vi "1_Sin(x)(Training).vi"() -> ()   [LabVIEW 2020]
uses:
  <vilib>/Ngene/Deep Learning Toolkit/Toolkit/NN_Train/Controls/NN_Train_Params.ctl
  <vilib>/Ngene/Deep Learning Toolkit/Toolkit/NN_Train/Controls/NN_Train_Optimizer.ctl
  <vilib>/Ngene/Deep Learning Toolkit/Toolkit/NN_Train/Controls/NN_Train_Data_Sampling.ctl
  <vilib>/Ngene/Deep Learning Toolkit/Toolkit/NN_Train/Controls/NN_LR_Policy_Cfg.ctl
  <vilib>/Ngene/Deep Learning Toolkit/Toolkit/NN_Train/Controls/NN_LR_Policy_Type.ctl
  <vilib>/Ngene/Deep Learning Toolkit/Toolkit/NN_Train/Controls/NN_Train_Session_Data.ctl
  <vilib>/Ngene/Deep Learning Toolkit/Toolkit/NN_Layers/Layers/Input/Controls/NN_Layer_Config(Input1D).ctl
  <vilib>/Ngene/Deep Learning Toolkit/Toolkit/NN_Data/Controls/NN_Data_type.ctl
  <vilib>/Ngene/Deep Learning Toolkit/Toolkit/NN_Network/Controls/NN_Save_Before_Destroy_Options.ctl
  <vilib>/Ngene/Deep Learning Toolkit/Toolkit/NN_Network/Controls/NN_Device.ctl
  <vilib>/Ngene/Deep Learning Toolkit/Toolkit/NN_Layers/Layers/FC/Controls/NN_Layer_Config(FC).ctl
  <vilib>/Ngene/Deep Learning Toolkit/Toolkit/NN_Layers/Layers/BatchNorm/Controls/NN_BN_Params.ctl
  <vilib>/Ngene/Deep Learning Toolkit/Toolkit/NN_Activations/Controls/NN_Activation_Type.ctl
  <vilib>/Ngene/Deep Learning Toolkit/Toolkit/NN_Layers/Controls/NN_Layer_Init_Params.ctl
  <vilib>/Ngene/Deep Learning Toolkit/Toolkit/NN_Layers/Controls/NN_Layer_Weight_Init_Type.ctl
  <vilib>/Ngene/Deep Learning Toolkit/Toolkit/NN_Data/API/DataSet/DataSet_Types/NN_DataSet(In1D_Out1D).ctl
  <vilib>/Ngene/Deep Learning Toolkit/Toolkit/NN_Data/Controls/DataRef_Types/2D/NN_Data_ref(2D_SGL).ctl
  <vilib>/Analysis/1siggen.llb/Ramp Pattern by Samples.vi
  <vilib>/Ngene/Deep Learning Toolkit/Toolkit/NN_Layers/Layers/Input/NN_Layer_Create(Input1D).vi
  <vilib>/Ngene/Deep Learning Toolkit/Toolkit/NN_Layers/Layers/FC/NN_Layer_Create(FC).vi
  <vilib>/Ngene/Deep Learning Toolkit/Toolkit/NN_Train/Loss_Functions/NN_Set_Loss(MSE).vi
  <vilib>/Ngene/Deep Learning Toolkit/Toolkit/NN_Data/subVIs/Get_Data_Vals/2D/NN_Data_Get_ValByRef(2D_SGL).vi
  <vilib>/Ngene/Deep Learning Toolkit/Toolkit/NN_Network/subVIs/NN_Predict/NN_Predict(In1D_Out1D).vi
  <vilib>/Ngene/Deep Learning Toolkit/Toolkit/NN_Train/Eval_Loss/NN_Eval_Test_Error_Loss/NN_Eval(In1D_Out1D).vi
  <vilib>/Ngene/Deep Learning Toolkit/Toolkit/Deep_Learning_Toolkit_by_Ngene.lvlib
  <vilib>/Analysis/NI_AALBase.lvlib
panel:
  out "Loop Time":dbl=0.0014889000000266606 format="%#_4p"
  out "Test Loss":sgl=6.473779e-05
  out "Training Loss":sgl=6.795796e-05
  in  "Stop":bool
  out "Loss Chart":cluster{"Loss":sgl, "Test Loss":sgl}(graph)={"Loss"=6.795796e-05, "Test Loss"=6.473779e-05}
  in  "# of Sine Cycles":dbl=4.0
  out "Sin(x): Predictions vs Ground Truths":sgl[][](graph)
  in  "Eval?":bool
  out "Session Data":T1={"Epochs"=1922.368, "Tot_Iter"=30037, "LR"=1.953125e-05, "LR_iter"=30038}
  in  "LR_Decay_Params":T2={"Policy_Type"=enum."Step", "LR0"=0.01, "k"=200.0, "WarmUp_Policy"=enum."Ramp", "WarmUp_Iter"=100, "WarmUp_Ratio"=10.0} {"WarmUp_Ratio" min=1; "WarmUp_Iter" min=1; "LR0" format="%.7f"}
  in  "NN_Train_Params":T4={"Optimizer"=enum."Adam", "Beta_1"=0.9, "Beta_2"=0.999, "Weight Decay(L1)"=1e-08, "Weight Decay(L2)"=1e-08, "Data_Sampling"=enum."Random"}
  # "Overview: Demonstrates the usage of DeepLTK (Deep Learning Toolkit for LabVIEW) for solving a simple regression problem of modeling sin(x) function.\nRequirements: DeepLTK - Deep Learning Toolkit for LabVIEW (https://www.ngene.co/deep-learning-toolkit-for-labview)\nInstructions:\n1. Run the VI with default configurations.\n2. Observe how the training loss is decreasing.\n3. Periodically press \"Eval?\" button to observe \"Test Loss\" and performance of the model on Test Dataset\n4. Press \"Stop\" when \"Test Loss\" is is not decreasing. ~1500 epochs\nMore Examples:  https://github.com/ngenehub/deepltk_examples"
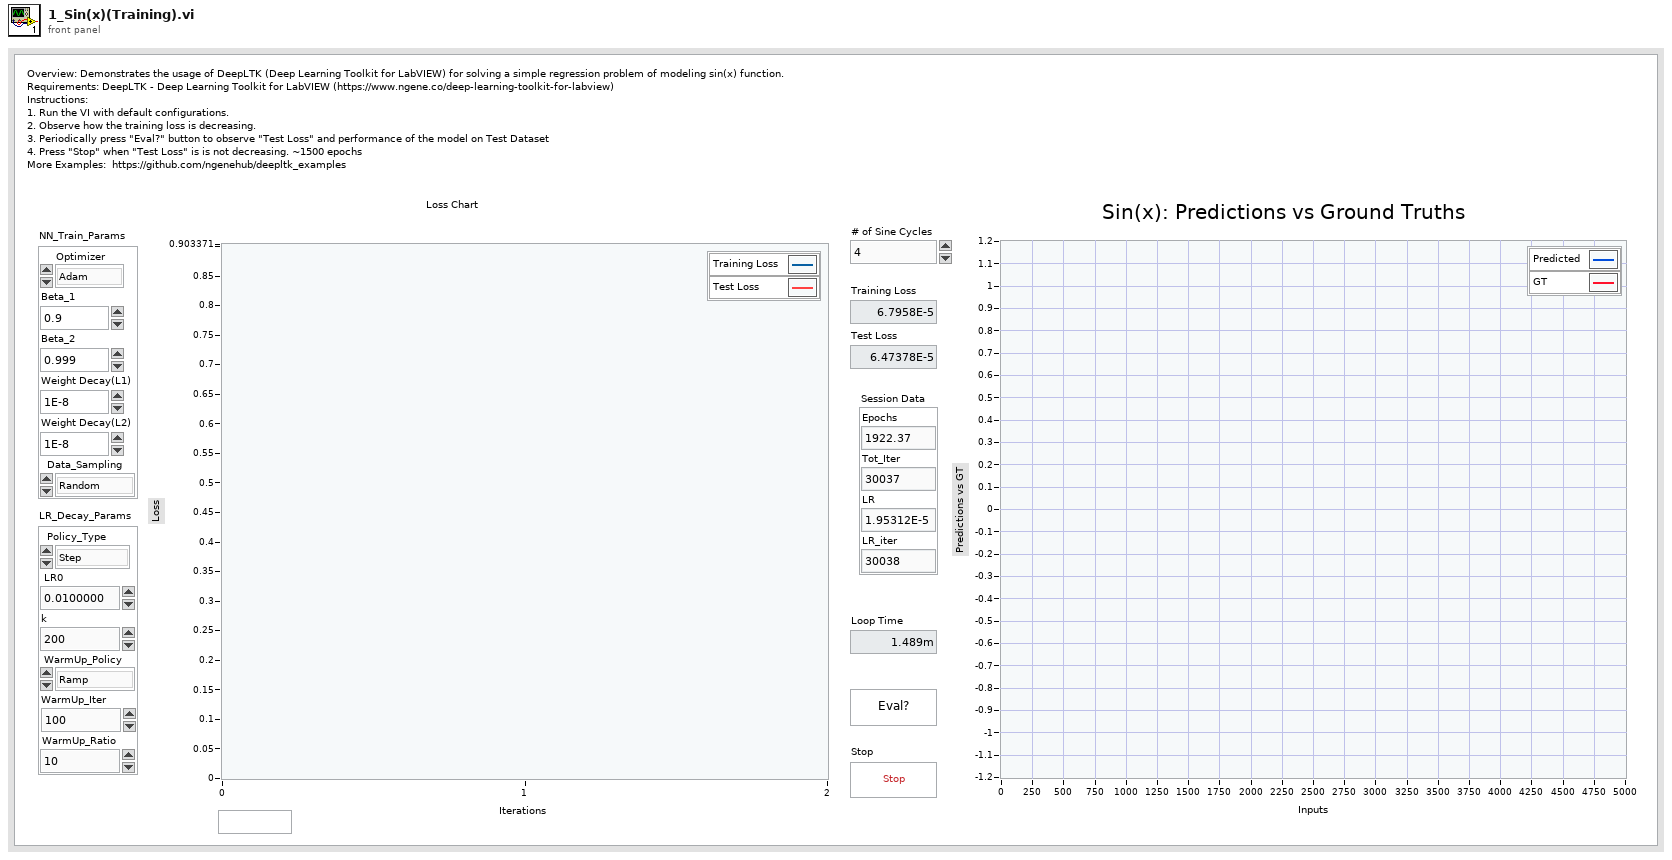
[diagram p1: front panel]
types:
  T1 = typedef "Deep_Learning_Toolkit_by_Ngene.lvlib/NN_Train_Session_Data.ctl" = cluster{"Epochs":sgl, "Tot_Iter":i32, "LR":sgl, "LR_iter":i32}
  T2 = typedef "Deep_Learning_Toolkit_by_Ngene.lvlib/NN_LR_Policy_Cfg.ctl" = cluster{"Policy_Type":T3, "LR0":dbl, "k":sgl, "WarmUp_Policy":enum16{"Step", "Ramp"}, "WarmUp_Iter":i32, "WarmUp_Ratio":sgl}
  T3 = typedef "Deep_Learning_Toolkit_by_Ngene.lvlib/NN_LR_Policy_Type.ctl" = enum16{"Manual", "Step", "Exp", "1/t"}
  T4 = typedef "Deep_Learning_Toolkit_by_Ngene.lvlib/NN_Train_Params.ctl" = cluster{"Optimizer":T5, "Beta_1":sgl, "Beta_2":sgl, "Weight Decay(L1)":sgl, "Weight Decay(L2)":sgl, "Data_Sampling":T6}
  T5 = typedef "Deep_Learning_Toolkit_by_Ngene.lvlib/NN_Train_Optimizer.ctl" = enum16{"SGD", "Adam", "Adagrad", "Adadelta", "RMSProp", "Nesterov"}
  T6 = typedef "Deep_Learning_Toolkit_by_Ngene.lvlib/NN_Train_Data_Sampling.ctl" = enum16{"Random", "Sequential"}
  T7 = typedef "Deep_Learning_Toolkit_by_Ngene.lvlib/NN_Layer_Config(FC).ctl" = cluster{"Name":string, "Size":i32, "BN":bool, "BN_Params":T8, "Activation":T9, "Has Bias?":bool, "Init_Params":T10, "Custom_Params":string}
  T8 = typedef "Deep_Learning_Toolkit_by_Ngene.lvlib/NN_BN_Params.ctl" = cluster{"epsilon":sgl, "momentum":sgl}
  T9 = typedef "Deep_Learning_Toolkit_by_Ngene.lvlib/NN_Activation_Type.ctl" = enum16{"Sigmoid", "ReLU", "LReLU", "ReLU6", "GELU", "tanh", "Swish", "Mish", "None"}
  T10 = typedef "Deep_Learning_Toolkit_by_Ngene.lvlib/NN_Layer_Init_Params.ctl" = cluster{"Init_Type":T11, "Value":sgl}
  T11 = typedef "Deep_Learning_Toolkit_by_Ngene.lvlib/NN_Layer_Weight_Init_Type.ctl" = enum16{"Const", "Uniform", "Gaussian", "Xavier"}
  T12 = typedef "Deep_Learning_Toolkit_by_Ngene.lvlib/NN_DataSet(In1D_Out1D).ctl" = cluster{"Inputs Ref.":variant, "Outputs Ref.":T13, "Dims_In":i32, "Dataset_Size":i32, "Dims_Out":i32, "Labels":string[], "File Paths":path[], "Custom_Data":variant}
  T13 = typedef "Deep_Learning_Toolkit_by_Ngene.lvlib/NN_Data_ref(2D_SGL).ctl" = refnum<data-value>
  T14 = typedef "Deep_Learning_Toolkit_by_Ngene.lvlib/NN_Device.ctl" = enum16{"CPU", "GPU"}
  T15 = typedef "Deep_Learning_Toolkit_by_Ngene.lvlib/NN_Save_Before_Destroy_Options.ctl" = cluster{"CFG?":bool, "Weights?":bool, "Render?":bool}
  T16 = typedef "Deep_Learning_Toolkit_by_Ngene.lvlib/NN_Layer_Config(Input1D).ctl" = cluster{"Name":string, "Size":i32, "Data_Type":T17, "Shift":sgl, "Scale":sgl}
  T17 = typedef "Deep_Learning_Toolkit_by_Ngene.lvlib/NN_Data_type.ctl" = enum16{"I8", "U8", "I16", "U16", "U32 ARGB", "SGL"}
  T18 = typedef "Deep_Learning_Toolkit_by_Ngene.lvlib/NN.ctl" = cluster{"Name":string, "No of Layers":i32, "mBatch":i32, "Layers":T19[], "Dimty":T20, "Dims_In":T21, "Dims_Out":T21, "Working_Dir":path, "Train?":bool, "Train_Params":T4, "LR_Update_Policy":T2, "Session Data":T1, "Ground_truth":T22, "NNg_hdls":T23, "NN_Device":T14, "GPU Id":i32, "Labels":string[], "Loss_Type":T24, "Loss_Cfg_Prms":variant, "NNG_WS":T25, "DryRun?":bool}
  T19 = typedef "Deep_Learning_Toolkit_by_Ngene.lvlib/NN_Layer_ref.ctl" = refnum<file>
  T20 = typedef "Deep_Learning_Toolkit_by_Ngene.lvlib/NN_In_Out_Dim-ty.ctl" = enum8{"In1D_Out1D", "In3D_Out1D", "In3D_Out3D", "In3D_OutBBox"}
  T21 = typedef "Deep_Learning_Toolkit_by_Ngene.lvlib/NN_Dims(C,H,W).ctl" = cluster{"C":i32, "H":i32, "W":i32}
  T22 = typedef "Deep_Learning_Toolkit_by_Ngene.lvlib/NN_Ground_truth.ctl" = cluster{"Y":variant}
  T23 = typedef "Deep_Learning_Toolkit_by_Ngene.lvlib/nng_cuda_handles.ctl" = cluster{"cudnn":u64, "cublas":u64, "stream":u64, "curand":u64}
  T24 = typedef "Deep_Learning_Toolkit_by_Ngene.lvlib/NN_Loss_Type.ctl" = enum16{"None", "MSE", "CrossEntropy", "YOLO_v2", "YOLO_v4"}
  T25 = typedef "Deep_Learning_Toolkit_by_Ngene.lvlib/NNG_WS.ctl" = cluster{"NNG_WS_Mem":T26, "Max_WS_Size":i64}
  T26 = typedef "Deep_Learning_Toolkit_by_Ngene.lvlib/NNg_WS_Mem_DVR.ctl" = refnum<data-value>
  T27 = typedef "Deep_Learning_Toolkit_by_Ngene.lvlib/NN_Eval_Params.ctl" = cluster{"Loss":sgl, "Error":sgl}
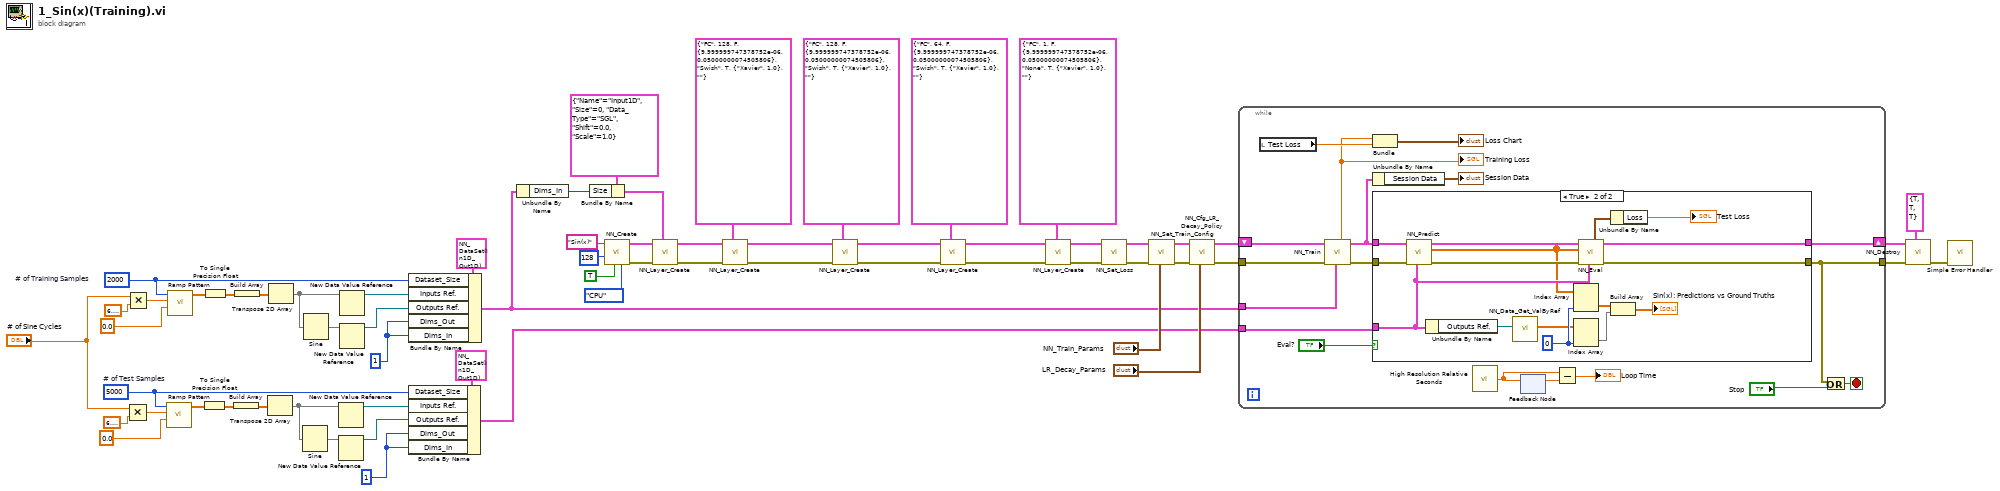
[diagram p0: block diagram]
diagram:
  w8 = 1 ("Dims_Out")
  w10 = 2000  # # of Training Samples
  w22 = 5000  # # of Test Samples
  w23 = 1 ("Dims_Out")
  n1 = Multiply(x="# of Sine Cycles", y=6.283185307179586) -> (x*y=w31:dbl)
  n2 = Multiply(x="# of Sine Cycles", y=6.283185307179586) -> (x*y=w17:dbl)
  n3 = call-poly <vilib>:"Ramp Pattern.vi"("start"=0.0, "end"=w31, "samples"=w22) -> ("Ramp Pattern"=w29:dbl[])  [unwired: 7 in, 1 out]
  n4 = call-poly <vilib>:"Ramp Pattern.vi"("start"=0.0, "end"=w17, "samples"=w10) -> ("Ramp Pattern"=w15:dbl[])  [unwired: 7 in, 1 out]
  n5 = To Single Precision Float(number=w29) -> (single precision float=w30:sgl[])
  n6 = To Single Precision Float(number=w15) -> (single precision float=w16:sgl[])
  n7 = Build Array(w30) -> (w28:sgl[][])
  n8 = Build Array(w16) -> (w14:sgl[][])
  n9 = Transpose 2D Array(2D array=w28) -> (transposed array=w27:sgl[][])
  n10 = Transpose 2D Array(2D array=w14) -> (transposed array=w13:sgl[][])
  n11 = Sine(x=w27) -> (sin(x)=w26:sgl[][])
  n12 = Sine(x=w13) -> (sin(x)=w12:sgl[][])
  n13 = New Data Value Reference(data value=w27) -> (data value reference=w34:refnum<data-value>)  [unwired: 1 in, 1 out]
  n14 = New Data Value Reference(data value=w26) -> (data value reference=w33:refnum<data-value>)  [unwired: 1 in, 1 out]
  n15 = New Data Value Reference(data value=w13) -> (data value reference=w20:refnum<data-value>)  [unwired: 1 in, 1 out]
  n16 = New Data Value Reference(data value=w12) -> (data value reference=w19:refnum<data-value>)  [unwired: 1 in, 1 out]
  n17 = Bundle By Name(cluster=T12 {"Inputs Ref."=variant(refnum<data-value> refnum), "Outputs Ref."=refnum, "Dims_In"=0, "Dataset_Size"=0, "Dims_Out"=0, "Labels"=[], "File Paths"=[], "Custom_Data"=variant} ("Dataset(In1D_Out1D)"), "Dataset_Size"=w22, "Inputs Ref."=w34, "Outputs Ref."=w33, "Dims_Out"=w23, "Dims_In"=w23) -> (w25:T12)
  n18 = Bundle By Name(cluster=T12 {"Inputs Ref."=variant(refnum<data-value> refnum), "Outputs Ref."=refnum, "Dims_In"=0, "Dataset_Size"=0, "Dims_Out"=0, "Labels"=[], "File Paths"=[], "Custom_Data"=variant} ("Dataset(In1D_Out1D)"), "Dataset_Size"=w10, "Inputs Ref."=w20, "Outputs Ref."=w19, "Dims_Out"=w8, "Dims_In"=w8) -> (w9:T12)
  n19 = Unbundle By Name(w9) -> ("Dims_In"=w40:i32)
  n20 = Bundle By Name(cluster=T16 {"Name"="Input1D", "Size"=0, "Data_Type"=enum."SGL", "Shift"=0.0, "Scale"=1.0} ("Input1D_Cfg"), "Size"=w40) -> (w56:T16)
  n21 = call <vilib>:"NN_Create.vi"("NN_Device"=NN_Device."CPU", "Train? (false)"=TRUE, "mBatch (1)"=128, "Name"="Sin(x)") -> ("error out"=w61:errorcluster, "NN out"=w62:T18)  [unwired: 6 in]
  n22 = call-poly <vilib>:"NN_Layer_Create.vi"("Input1D_Cfg"=w56, "error in (no error)"=w61, "NN in"=w62) -> ("error out"=w64:errorcluster, "NN out"=w63:T18)  [unwired: 6 in, 1 out]
  n23 = call-poly <vilib>:"NN_Layer_Create.vi"("FC_Cfg"=T7 {"Name"="FC", "Size"=128, "BN"=FALSE, "BN_Params"={"epsilon"=1e-05, "momentum"=0.05}, "Activation"=enum."Swish", "Has Bias?"=TRUE, "Init_Params"={"Init_Type"=enum."Xavier", "Value"=1.0}, "Custom_Params"=""}, "error in (no error)"=w64, "NN in"=w63) -> ("error out"=w37:errorcluster, "NN out"=w38:T18)  [unwired: 6 in, 1 out]
  n24 = call-poly <vilib>:"NN_Layer_Create.vi"("FC_Cfg"=T7 {"Name"="FC", "Size"=128, "BN"=FALSE, "BN_Params"={"epsilon"=1e-05, "momentum"=0.05}, "Activation"=enum."Swish", "Has Bias?"=TRUE, "Init_Params"={"Init_Type"=enum."Xavier", "Value"=1.0}, "Custom_Params"=""}, "error in (no error)"=w37, "NN in"=w38) -> ("error out"=w4:errorcluster, "NN out"=w5:T18)  [unwired: 6 in, 1 out]
  n25 = call-poly <vilib>:"NN_Layer_Create.vi"("FC_Cfg"=T7 {"Name"="FC", "Size"=64, "BN"=FALSE, "BN_Params"={"epsilon"=1e-05, "momentum"=0.05}, "Activation"=enum."Swish", "Has Bias?"=TRUE, "Init_Params"={"Init_Type"=enum."Xavier", "Value"=1.0}, "Custom_Params"=""}, "error in (no error)"=w4, "NN in"=w5) -> ("error out"=w2:errorcluster, "NN out"=w3:T18)  [unwired: 6 in, 1 out]
  n26 = call-poly <vilib>:"NN_Layer_Create.vi"("FC_Cfg"=T7 {"Name"="FC", "Size"=1, "BN"=FALSE, "BN_Params"={"epsilon"=1e-05, "momentum"=0.05}, "Activation"=enum."None", "Has Bias?"=TRUE, "Init_Params"={"Init_Type"=enum."Xavier", "Value"=1.0}, "Custom_Params"=""}, "error in (no error)"=w2, "NN in"=w3) -> ("error out"=w42:errorcluster, "NN out"=w41:T18)  [unwired: 6 in, 1 out]
  n27 = call-poly <vilib>:"NN_Set_Loss.vi"("error in (no error)"=w42, "NN in"=w41) -> ("error out"=w43:errorcluster, "NN out"=w44:T18)  [unwired: 8 in]
  n28 = call <vilib>:"NN_Set_Train_Config.vi"("NN_Train_Params"="NN_Train_Params", "error in (no error)"=w43, "NN in"=w44) -> ("error out"=w49:errorcluster, "NN out"=w54:T18)  [unwired: 7 in]
  n29 = call <vilib>:"NN_Cfg_LR_Decay_Policy.vi"("LR_Decay_Params"="LR_Decay_Params", "error in (no error)"=w49, "NN in"=w54) -> ("error out"=w48:errorcluster, "NN out"=w50:T18)  [unwired: 7 in]
  n30 = while {
    tunnel: w48 -> [w81]
    tunnel: w9 -> [w66]
    shift-right: [w77] -> w52
    shift-left: w50 -> [w82]
    tunnel: [w73] -> w51
    tunnel: w25 -> [w65]
    stop <- w80 stop-if-true
    n31 = local read "Test Loss"() -> (w74:sgl)
    n32 = call <vilib>:"NN_Train.vi"("Train Dataset"=w66, "error in (no error)"=w81, "NN in"=w82) -> ("error out"=w76:errorcluster, "NN out"=w79:T18, "Loss"=w67:sgl)  [unwired: 3 in, 3 out]
    "Training Loss" <- w67
    n33 = Bundle("Loss"=w67, "Test Loss"=w74) -> (→"Loss Chart":cluster{"Loss":sgl, "Test Loss":sgl})  [unwired: 1 in]
    n34 = Unbundle By Name(w79) -> ("Session Data"=→"Session Data":T1)
    n35 = case shown="True" "Eval?" {
      tunnel: w79 -> [w84 w96]
      tunnel: [w84 w100] -> w77
      tunnel: w76 -> [w83 w95]
      tunnel: [w83 w99] -> w73
      tunnel: w65 -> [_ w94]
      frame False {
      }
      frame True {
        w91 = 0 ("disabled index (col)")
        n36 = call-poly <vilib>:"NN_Predict.vi"("Dataset"=w94, "error in (no error)"=w95, "NN in"=w96) -> ("error out"=w97:errorcluster, "Predictions"=w92:sgl[][], "NN out"=w98:T18)  [unwired: 6 in]
        n37 = Unbundle By Name(w94) -> ("Outputs Ref."=w93:T13)
        n38 = call-poly <vilib>:"NN_Data_Get_ValByRef.vi"("DVR(2D_SGL)"=w93) -> ("Value(2D_SGL)"=w88:sgl[][])  [unwired: 7 in, 1 out]
        n39 = Index Array(array=w92, index (col)=w91) -> (element=w87:sgl[])  [unwired: 1 in]
        n40 = Index Array(array=w88, index (col)=w91) -> (element=w90:sgl[])  [unwired: 1 in]
        n41 = call-poly <vilib>:"NN_Eval.vi"("Dataset"=w94, "error in (no error)"=w97, "Predictions"=w92, "NN in"=w98) -> ("error out"=w99:errorcluster, "NN out"=w100:T18, "NN_Eval_Params"=w86:T27)  [unwired: 4 in, 1 out]
        n42 = Unbundle By Name(w86) -> ("Loss"=→"Test Loss":sgl)
        n43 = Build Array(w87, w90) -> (→"Sin(x): Predictions vs Ground Truths":sgl[][])
      }
    }
    n44 = call <vilib>:"High Resolution Relative Seconds.vi"() -> ("relative seconds"=w72:dbl)
    n45 = feedback-in #1(w72) -> ()
    n46 = feedback #1() -> (w71:dbl)  [unwired: 1 in]
    n47 = Subtract(x=w72, y=w71) -> (x-y=→"Loop Time":dbl)
    n48 = Or(x=w73, y="Stop") -> (x .or. y?=w80:bool)
  }
  n49 = call <vilib>:"NN_Destroy.vi"("Save (T, T, T)"=T15 {"CFG?"=TRUE, "Weights?"=TRUE, "Render?"=TRUE}, "error in (no error)"=w51, "NN in"=w52) -> ("error out"=w1:errorcluster)  [unwired: 7 in, 1 out]
  n50 = call <vilib>:"Simple Error Handler.vi"("error in (no error)"=w1) -> ()  [unwired: 4 in, 5 out]
